vi "DAC_Measurement_Specs.vi"(0 "DAC Device Tests":T1, 11 "Error In":errorcluster) -> (15 "Error Out":errorcluster)   [LabVIEW 2026, in "Core.lvlib"]
doc: "Provides selection and configuration of DAC tests and loads the corresponding test specification parameters."
uses:
  Core.lvlib
  TypeDefs/DAC/Enum_DAC_Tests.ctl
  TypeDefs/Enum_Events.ctl
  TypeDefs/Enum_Event_Options.ctl
panel:
  # "Instructions:\n-> Choose a DAC test from the dropdown.\n\n-> Enter the required test specifications displayed in the Test Specs section."
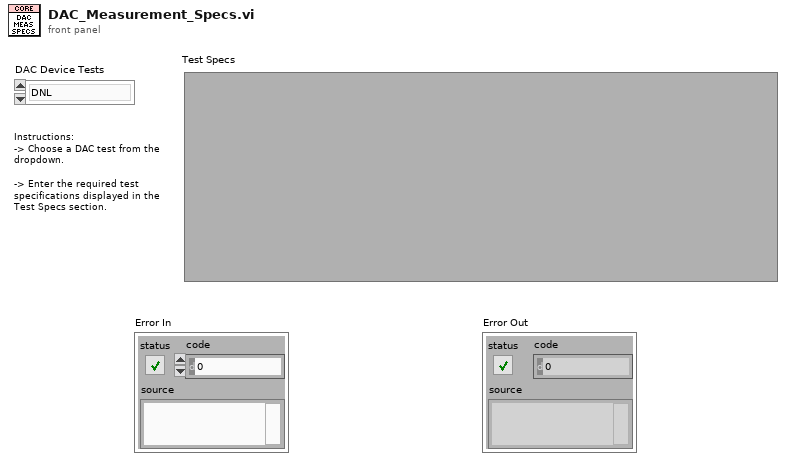
[diagram p1: front panel]
types:
  T1 = typedef "Core.lvlib/Enum_DAC_Tests.ctl" = enum16{"DNL", "INL"}
  T2 = typedef "Core.lvlib/Enum_Events.ctl" = enum16{"Stop All", "Stop Subpanel", "Stop Test Spec", "Stop Result"}
  T3 = typedef "Core.lvlib/Enum_Event_Options.ctl" = enum16{"Create", "Generate", "Event Ref", "Destroy"}
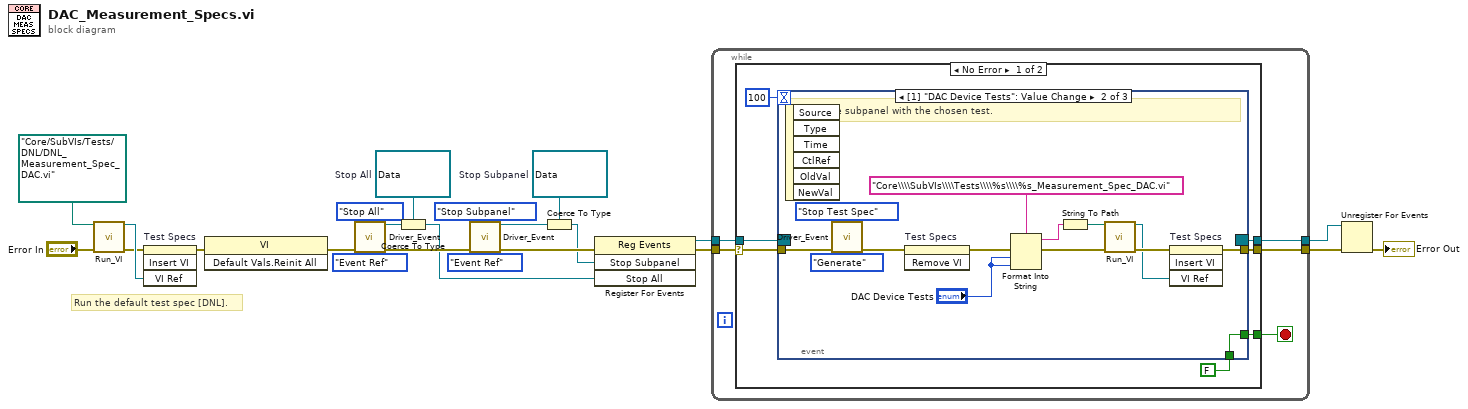
[diagram p0: block diagram]
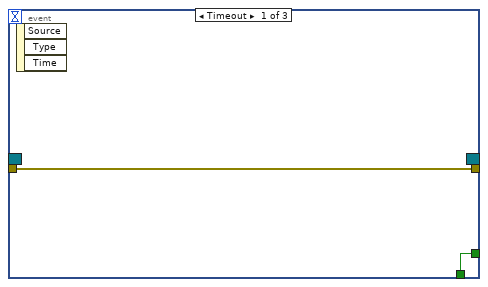
[diagram p2: hidden frame]
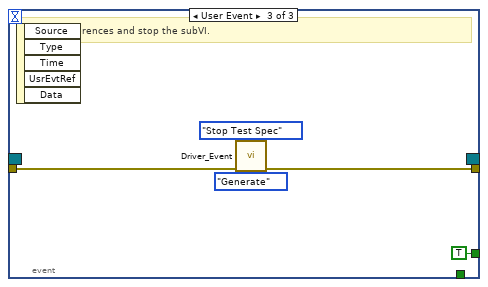
[diagram p3: hidden frame]
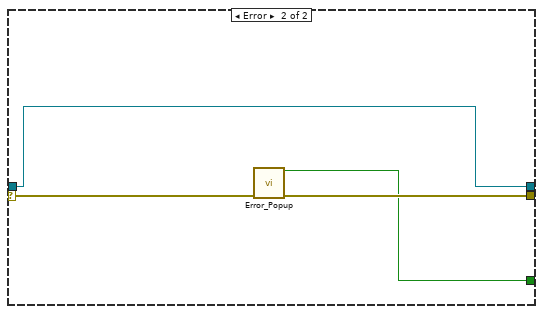
[diagram p4: hidden frame]
diagram:
  w6 = refnum<user-event> refnum  # Stop All
  w16 = refnum<user-event> refnum  # Stop Subpanel
  # "Run the default test spec [DNL]."
  n1 = call "Run_VI.vi"("Path"=path "Core/SubVIs/Tests/DNL/DNL_Measurement_Spec_DAC.vi", "Error In"="Error In") -> ("VI Refnum"=w4:refnum<vi>, "Error Out"=w2:errorcluster)  [unwired: 12 in]
  n2 = invoke on="Test Specs" class="SubPnl" method="Insert VI"(error in=w2, "VI Ref"=w4) -> (error out=w1:errorcluster)  [unwired: 2 in, 3 out]
  n3 = invoke class="VI" method="Default Vals.Reinit All"(error in=w1) -> (error out=w11:errorcluster)  [unwired: 2 in, 2 out]
  n4 = call "Driver_Event.vi"("Event"=Enum_Events."Stop All", "Error In"=w11, "Event Operation"=Enum_Event_Options."Event Ref") -> ("Event Ref"=w8:refnum<user-event>, "Error Out"=w12:errorcluster)  [unwired: 11 in]
  n5 = Coerce To Type(0:w8, 1:w6) -> (2:w7:refnum<user-event>)
  n6 = call "Driver_Event.vi"("Event"=Enum_Events."Stop Subpanel", "Error In"=w12, "Event Operation"=Enum_Event_Options."Event Ref") -> ("Event Ref"=w22:refnum<user-event>, "Error Out"=w21:errorcluster)  [unwired: 11 in]
  n7 = Coerce To Type(0:w22, 1:w16) -> (2:w13:refnum<user-event>)
  n8 = register-events(error in=w21, w13, w7) -> (reference out=w19:refnum<event-registration>, error out=w20:errorcluster)  [unwired: 1 in]
  n9 = while {
    tunnel: w20 -> [w27]
    tunnel: [w28] -> w23
    tunnel: w19 -> [w26]
    tunnel: [w25] -> w17
    stop <- w24 stop-if-true
    n10 = case shown="No Error" w27 {
      selector: w27 -> [w34 w60]
      tunnel: [w35 w59] -> w28
      tunnel: w26 -> [w32 w58]
      tunnel: [w31 w58] -> w25
      tunnel: [w30 w57] -> w24
      frame No Error {
        n11 = event shown="[1] \"DAC Device Tests\": Value Change" {
          selector: w32 -> [_ _ _]
          dyn-events: [_ _ _] -> w31
          timeout: 100 -> [_ _ _]
          tunnel: [w36 w40 w52] -> w35
          tunnel: w34 -> [w36 w50 w53]
          tunnel: [w37 w51 TRUE] -> w30
          tunnel: FALSE -> [w37 w51 _]
          event Timeout {
            n12 = event-data() -> ()  [unwired: 1 in, 3 out]
          }
          event Value Change {
            # "Update the subpanel with the chosen test."
            n13 = event-data() -> ()  [unwired: 1 in, 6 out]
            n14 = call "Driver_Event.vi"("Event"=Enum_Events."Stop Test Spec", "Error In"=w50, "Event Operation"=Enum_Event_Options."Generate") -> ("Error Out"=w39:errorcluster)  [unwired: 11 in, 1 out]
            n15 = invoke on="Test Specs" class="SubPnl" method="Remove VI"(error in=w39) -> (error out=w38:errorcluster)  [unwired: 2 in, 2 out]
            n16 = Format Into String(format string="Core\\\\SubVIs\\\\Tests\\\\%s\\\\%s_Measurement_Spec_DAC.vi", error in=w38, "DAC Device Tests", "DAC Device Tests") -> (resulting string=w42:string, error out=w46:errorcluster)  [unwired: 1 in]
            n17 = String To Path(string=w42) -> (path=w41:path)
            n18 = call "Run_VI.vi"("Path"=w41, "Error In"=w46) -> ("VI Refnum"=w43:refnum<vi>, "Error Out"=w47:errorcluster)  [unwired: 12 in]
            n19 = invoke on="Test Specs" class="SubPnl" method="Insert VI"(error in=w47, "VI Ref"=w43) -> (error out=w40:errorcluster)  [unwired: 2 in, 3 out]
          }
          event User Event {
            # "Close all references and stop the subVI."
            n20 = event-data() -> ()  [unwired: 1 in, 5 out]
            n21 = call "Driver_Event.vi"("Event"=Enum_Events."Stop Test Spec", "Error In"=w53, "Event Operation"=Enum_Event_Options."Generate") -> ("Error Out"=w52:errorcluster)  [unwired: 11 in, 1 out]
          }
        }
      }
      frame Error {
        n22 = call "Error_Popup.vi"("Error In"=w60) -> ("Stop?"=w57:bool, "Error Out"=w59:errorcluster)  [unwired: 13 in]
      }
    }
  }
  n23 = Unregister For Events(event registration refnum=w17, error in=w23) -> (error out=→"Error Out":errorcluster)
